vi "Create.vi"(8 "error in (no error)":errorcluster, 11 "CIFPlugin in":refnum<class "CAN_Reader_NIXNET_Plugin.lvclass">) -> (0 "error out":errorcluster, 3 "CIFPlugin out":refnum<class "CAN_Reader_NIXNET_Plugin.lvclass">)   [LabVIEW 2021, in "CAN_Reader_NIXNET_Plugin.lvclass"]
uses:
  CAN_Reader_NIXNET_Plugin.lvclass
  C:/Program Files/National Instruments/LabVIEW 2021/vi.lib/CIF Foundation/CIF Core/CIFCore/Class/CIFCorePlugin.lvclass
  <vilib>/CIF Foundation/CIF Core/CIFCore/Common/Typedef/Timing Overrides.ctl
  <vilib>/CIF Foundation/CIF U8 Array Monitor gRPC/U8_Array_Monitor_gRPC/CIFU8ArrayMonitorUtilities/Typedef/U8 Array.ctl
  <vilib>/CIF Foundation/CIF Channels Core/CIFChannels/CIFChannels.lvclass
  CAN_Reader_NIXNET_Plugin.lvclass/CAN_Reader_NIXNET_Plugin.ctl
  <vilib>/CIF Foundation/CIF Core/CIFCore/Class/CIFCorePlugin.lvclass/CIFCorePlugin.ctl
  <vilib>/CIF Foundation/CIF Core/CIFCore/Class/Accessors/Read Running Internal Data.vi
  <vilib>/CIF Foundation/CIF Core/CIFCore/Class/Accessors/Write Timing Override.vi
  <vilib>/CIF Foundation/CIF Core/CIFCore/Class/Accessors/Write Running Internal Data.vi
  Common/CAN_Reader_NIXNET_Common.lvlib
  <vilib>/CIF Foundation/CIF Core/CIFCore/Class/CIFCorePlugin.lvclass
  <vilib>/CIF Foundation/CIF Core/CIFCore/Common/CIFCoreCommon.lvlib
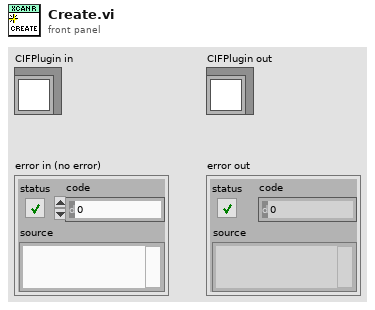
[diagram p1: front panel]
types:
  T1 = typedef "CIFCoreCommon.lvlib/Timing Overrides.ctl" = cluster{"Override Timing":bool, "Skip Sleep":bool, "Period (s)":dbl}
  T2 = typedef "U8 Array.ctl" = cluster{"Timestamp":i64, "U8 Array":u8[]}
  T3 = typedef "ChannelRegistrar.lvlib/Channel Definition.ctl" = cluster{"Name":string, "Direction":T4, "Type":T5, "Custom Config Data":u8[]}
  T4 = typedef "ChannelCommon.lvlib/Direction.ctl" = enum8{"Publisher", "Subscriber"}
  T5 = typedef "ChannelRegistrar.lvlib/Registered Channel Types.ctl" = enum8{"Custom", "Double_Tag", "I64_Tag", "U64_Tag", "U8_FIFO", "CAN_FIFO", "L2Enet_FIFO", "DAQ_FIFO", "Universal_FIFO", "String_Tag"}
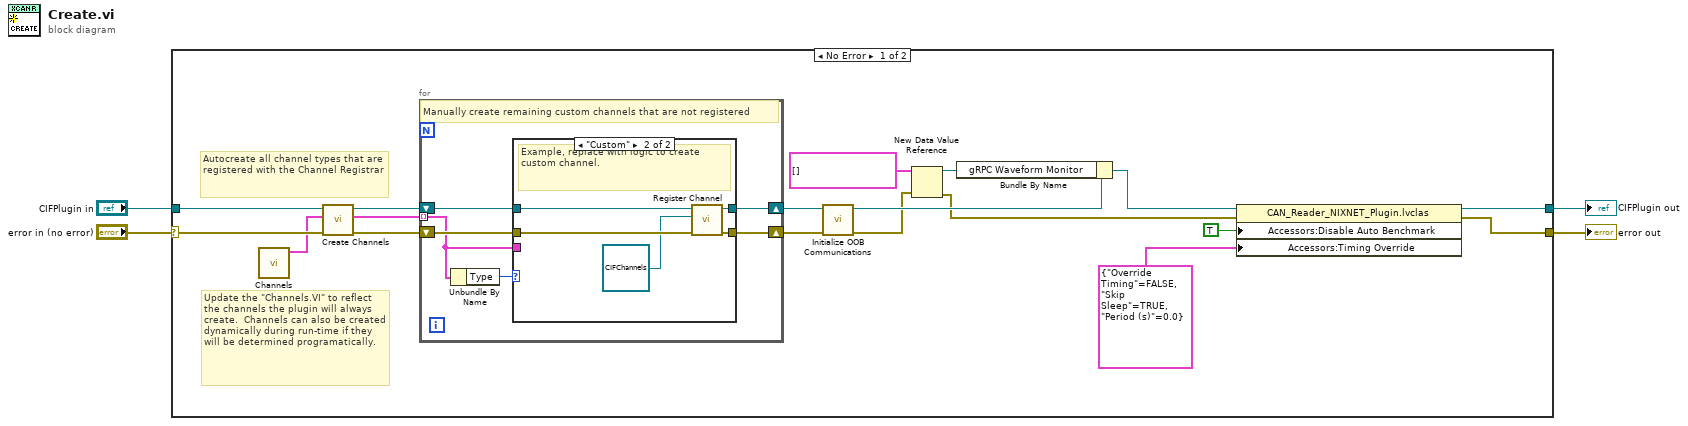
[diagram p0: block diagram]
diagram:
  n1 = case shown="No Error" "error in (no error)" {
    selector: "error in (no error)" -> [w21 w37]
    tunnel: [w5 w37] -> w1
    tunnel: [w6 w36] -> w2
    tunnel: "CIFPlugin in" -> [w22 w36]
    frame No Error {
      # "Update the \"Channels.VI\" to reflect the channels the plugin will always create.  Channels can also be created dynamically during run-time if they will be determined programatically."
      # "Autocreate all channel types that are registered with the Channel Registrar"
      n2 = call "Channels.vi"() -> ("Channels to Create"=w20:T3[])  [unwired: 10 in, 1 out]
      n3 = call <vilib>:"Create Channels.vi"("error in (no error)"=w21, "Channels to Create in"=w20, "CIFCorePlugin in"=w22) -> ("error out"=w17:errorcluster, "Channels to Create out"=w19:T3[], "CIFCorePlugin out"=w18:refnum<class "CAN_Reader_NIXNET_Plugin.lvclass">)  [unwired: 6 in]
      n4 = for {
        tunnel: w19 -> [w23] mode=indexing
        shift-right: [w26] -> w16
        shift-left: w18 -> [w28]
        shift-right: [w25] -> w15
        shift-left: w17 -> [w27]
        # "Manually create remaining custom channels that are not registered"
        n5 = Unbundle By Name(w23) -> ("Type"=w24:T5)
        n6 = case shown="\"Custom\"" w24 {
          tunnel: w28 -> [w30 w35]
          tunnel: w27 -> [w29 w34]
          tunnel: [w30 w33] -> w26
          tunnel: [w29 w32] -> w25
          tunnel: w23 -> [_ _]
          frame Default {
          }
          frame "Custom" {
            # "Example, replace with logic to create custom channel."
            n7 = call <vilib>:"Register Channel.vi"("error in (no error)"=w34, "Channel"=refnum<class "CIFChannels.lvclass"> refnum, "CIFCorePlugin in"=w35) -> ("error out"=w32:errorcluster, "CIFCorePlugin out"=w33:refnum<class "CAN_Reader_NIXNET_Plugin.lvclass">)  [unwired: 7 in]
          }
        }
      }
      n8 = call "Initialize OOB Communications.vi"("error in (no error)"=w15, "CIFPlugin in"=w16) -> ("error out"=w10:errorcluster, "CIFPlugin out"=w14:refnum<class "CAN_Reader_NIXNET_Plugin.lvclass">)  [unwired: 8 in]
      n9 = New Data Value Reference(data value=T2[] [] ("CIF U8 Array in"), error in=w10) -> (data value reference=w12:refnum<data-value>, error out=w9:errorcluster)
      n10 = Bundle By Name(cluster=w14, "gRPC Waveform Monitor"=w12) -> (w13:refnum<class "CAN_Reader_NIXNET_Plugin.lvclass">)
      n11 = property class="CAN_Reader_NIXNET_Plugin.lvclas"(reference=w13, error in=w9, "Accessors:Disable Auto Benchmark"=TRUE ("Disable Auto Benchmark"), "Accessors:Timing Override"=T1 {"Override Timing"=FALSE, "Skip Sleep"=TRUE, "Period (s)"=0.0} ("Timing Override")) -> (reference out=w6:refnum<class "CAN_Reader_NIXNET_Plugin.lvclass">, error out=w5:errorcluster)
    }
    frame Error {
    }
  }
  "CIFPlugin out" <- w2
  "error out" <- w1
